vi "GenerateXYArmPathPolygon.vi"(1 "PointSpacing (in)":dbl, 2 "EndPoint":T1, 3 "StartPoint":T1) -> (0 "XYPathPoints":T1[](array[typedef]))   [LabVIEW 2017]
uses:
  ArgosLib/Path Planning/TypeDefs/Point2D.ctl
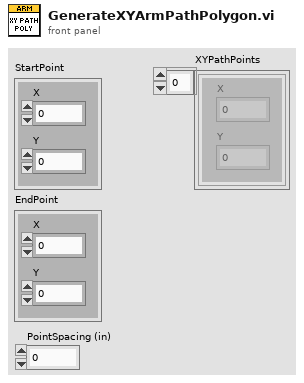
[diagram p1: front panel]
types:
  T1 = typedef "Point2D.ctl" = cluster{"X":dbl, "Y":dbl}
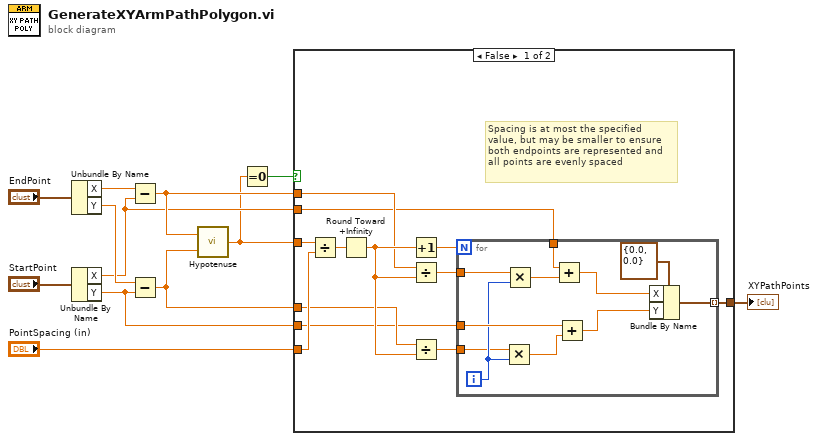
[diagram p0: block diagram]
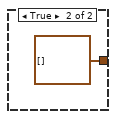
[diagram p2: hidden frame]
diagram:
  n1 = Unbundle By Name("EndPoint") -> ("X"=w7:dbl, "Y"=w6:dbl)
  n2 = Unbundle By Name("StartPoint") -> ("X"=w5:dbl, "Y"=w4:dbl)
  n3 = Subtract(x=w7, y=w5) -> (x-y=w11:dbl)
  n4 = Subtract(x=w6, y=w4) -> (x-y=w10:dbl)
  n5 = call "Hypotenuse.vi"("Y"=w10, "X"=w11) -> ("Hypotenuse"=w2:dbl)
  n6 = Equal To 0?(x=w2) -> (x = 0?=w1:bool)
  n7 = case shown="False" w1 {
    tunnel: "PointSpacing (in)" -> [w24 _]
    tunnel: w11 -> [w19 _]
    tunnel: w10 -> [w18 _]
    tunnel: w5 -> [w17 _]
    tunnel: w4 -> [w16 _]
    tunnel: [w15 T1[] []] -> w3
    tunnel: w2 -> [w13 _]
    frame False {
      # "Spacing is at most the specified\nvalue, but may be smaller to ensure\nboth endpoints are represented and\nall points are evenly spaced"
      n8 = Divide(x=w13, y=w24) -> (x/y=w23:dbl)
      n9 = Round Toward +Infinity(x=w23) -> (ceil(x): smallest int >= x=w22:dbl)
      n10 = Increment(x=w22) -> (x+1=w14:dbl)
      n11 = Divide(x=w19, y=w22) -> (x/y=w20:dbl)
      n12 = Divide(x=w18, y=w22) -> (x/y=w21:dbl)
      n13 = for {
        N: w14 -> [_]
        tunnel: w17 -> [w35]
        tunnel: w16 -> [w34]
        tunnel: w21 -> [w30]
        tunnel: w20 -> [w29]
        tunnel: [w25] -> w15 mode=indexing
        i -> [w32]
        n14 = Multiply(x=w30, y=w32) -> (x*y=w33:dbl)
        n15 = Multiply(x=w29, y=w32) -> (x*y=w31:dbl)
        n16 = Add(x=w35, y=w31) -> (x+y=w27:dbl)
        n17 = Add(x=w34, y=w33) -> (x+y=w26:dbl)
        n18 = Bundle By Name(cluster=T1 {"X"=0.0, "Y"=0.0} ("2DPoint"), "X"=w27, "Y"=w26) -> (w25:T1)
      }
    }
    frame True {
    }
  }
  "XYPathPoints" <- w3
